vi "validate line configuration.vi"(7 "EthernetIP configuration":refnum<class "EthernetIP configuration.lvclass">, 11 "line in":T1) -> (1 "valid?":bool, 2 "problem":string, 3 "line out":T1)   [LabVIEW 2013, in "EthernetIP editor node.lvclass"]
uses:
  EthernetIP editor node.lvclass
  table line.ctl
  channel/EthernetIP Channel.lvclass
  configuration/EthernetIP configuration.lvclass
  <vilib>/NI/Tag Bus/tag/Data Type.ctl
  channel/EthernetIP Channel.lvclass/EthernetIP Channel.ctl
  <vilib>/NI/Tag Bus/tag/tag descriptor.lvclass/tag descriptor.ctl
  <vilib>/NI/Tag Bus Module Framework/channel/TBM channel.lvclass/TBM channel.ctl
  configuration/EthernetIP configuration.lvclass/EthernetIP configuration.ctl
  channel/Read byte index.vi
  channel/Read Instance ID.vi
  configuration/read eip channels.vi
  configuration/Read assemblies.vi
  <vilib>/NI/Tag Bus/tag/read tag name.vi
  <vilib>/NI/Tag Bus Module Framework/channel/Read channel classification.vi
  <vilib>/NI/Tag Bus/tag/tag descriptor.lvclass
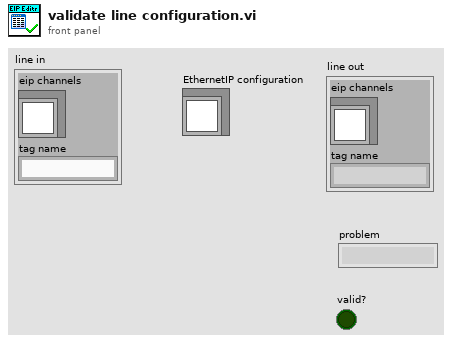
[diagram p1: front panel]
types:
  T1 = typedef "EthernetIP editor node.lvclass/table line.ctl" = cluster{"eip channels":refnum<class "EthernetIP Channel.lvclass">, "tag name":string}
  T2 = typedef "tag bus.lvlib/tag descriptor.lvclass/Data Type.ctl" = enum16{"Double", "Single", "I64", "I32", "I16", "I8", "U64", "U32", "U16", "U8", "Boolean", "String", "Array of Double", "Array of Single", "Array of I64", "Array of I32", "Array of I16", "Array of I8", "Array of U64", "Array of U32", "Array of U16", "Array of U8", "Array of Boolean", "Array of String"}
  T3 = typedef "TBM channel.lvclass/channel classification.ctl" = enum16{"input data", "output data", "processing parameter", "processing result"}
  T4 = typedef "EthernetIP configuration.lvclass/assembly definition.ctl" = cluster{"name":string, "Instance ID":u32, "Type":T5, "Size (elements)":u32, "big endian?":bool, "data type":T2}
  T5 = typedef "EthernetIP configuration.lvclass/assembly type.ctl" = enum32{"Producing", "Consuming"}
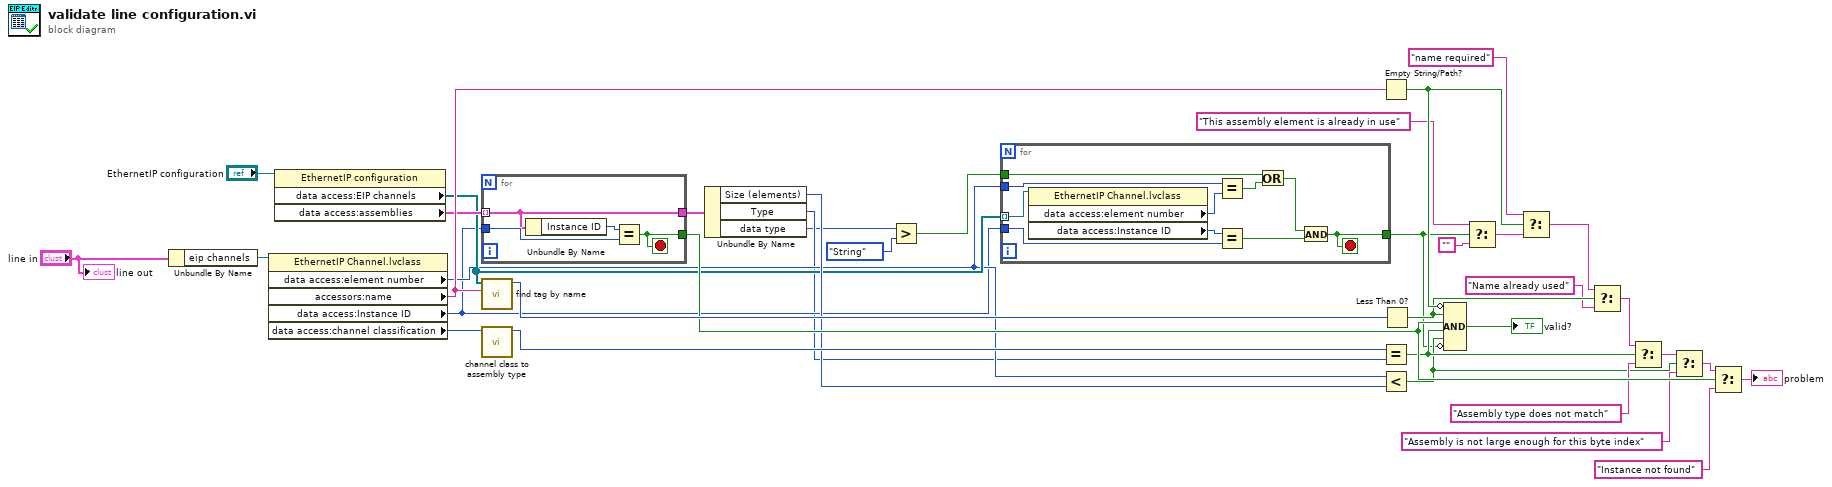
[diagram p0: block diagram]
diagram:
  n1 = Unbundle By Name("line in") -> ("eip channels"=w36:refnum<class "EthernetIP Channel.lvclass">)
  n2 = property class="EthernetIP Channel.lvclass"(reference=w36) -> ("data access:element number"=w10:i32, "accessors:name"=w34:string, "data access:Instance ID"=w9:u32, "data access:channel classification"=w23:T3)  [unwired: 1 in, 2 out]
  n3 = property class="EthernetIP configuration"(reference="EthernetIP configuration") -> ("data access:EIP channels"=w11:refnum<class "EthernetIP Channel.lvclass">[], "data access:assemblies"=w31:T4[])  [unwired: 1 in, 2 out]
  n4 = for {
    tunnel: w31 -> [w39] mode=indexing
    tunnel: w9 -> [w40]
    tunnel: [w39] -> w19
    tunnel: [w38] -> w24
    stop <- w38 stop-if-true
    n5 = Unbundle By Name(w39) -> ("Instance ID"=w41:u32)
    n6 = Equal?(x=w41, y=w40) -> (x = y?=w38:bool)
  }
  n7 = call <vilib>:"find tag by name.vi"("name"=w34, "tags in"=w11) -> ("index"=w32:i32)  [unwired: 9 in]
  n8 = call "channel class to assembly type.vi"("channel classification"=w23) -> ("assembly types"=w15:T5)  [unwired: 10 in]
  n9 = Unbundle By Name(w19) -> ("Size (elements)"=w13:u32, "Type"=w4:T5, "data type"=w3:T2)
  n10 = Greater?(x=w3, y=Data_Type."String") -> (0:w1:bool)
  n11 = for {
    tunnel: w11 -> [w51] mode=indexing
    tunnel: w10 -> [w49]
    tunnel: w9 -> [w47]
    tunnel: [w44] -> w5
    tunnel: w1 -> [w42]
    stop <- w44 stop-if-true
    n12 = property class="EthernetIP Channel.lvclass"(reference=w51) -> ("data access:element number"=w50:i32, "data access:Instance ID"=w48:u32)  [unwired: 1 in, 2 out]
    n13 = Equal?(x=w49, y=w50) -> (x = y?=w46:bool)
    n14 = Equal?(x=w48, y=w47) -> (x = y?=w45:bool)
    n15 = Or(x=w42, y=w46) -> (x .or. y?=w43:bool)
    n16 = And(x=w43, y=w45) -> (x .and. y?=w44:bool)
  }
  n17 = Empty String/Path?(string/path=w34) -> (empty?=w30:bool)
  n18 = Equal?(x=w15, y=w4) -> (x = y?=w14:bool)
  n19 = Less?(x=w10, y=w13) -> (x < y?=w12:bool)
  n20 = Less Than 0?(x=w32) -> (x < 0?=w29:bool)
  n21 = Compound Arithmetic op=AND(invert w30, w29, w24, w14, w12, invert w5) -> (→"valid?":bool)
  n22 = Select(t="This assembly element is already in use", s=w5, f="") -> (s? t:f=w7:string)
  n23 = Select(t="name required", s=w30, f=w7) -> (s? t:f=w28:string)
  n24 = Select(t=w28, s=w29, f="Name already used") -> (s? t:f=w18:string)
  n25 = Select(t=w18, s=w14, f="Assembly type does not match") -> (s? t:f=w20:string)
  n26 = Select(t=w20, s=w12, f="Assembly is not large enough for this byte index") -> (s? t:f=w17:string)
  n27 = Select(t=w17, s=w24, f="Instance not found") -> (s? t:f=→"problem":string)
  "line out" <- "line in"
